vi "remove Line Feed Character.vi"(8 "error in":errorcluster, 11 "Query String":string) -> (0 "error out":errorcluster, 3 "Line Feed Removed String":string)   [LabVIEW 2023, in "ANRITSU Call Box.lvlib"]
uses:
  ANRITSU Call Box.lvlib
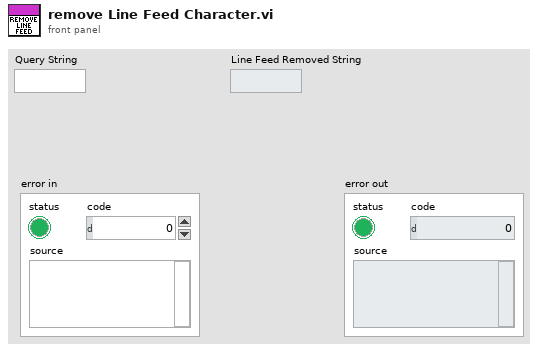
[diagram p1: front panel]
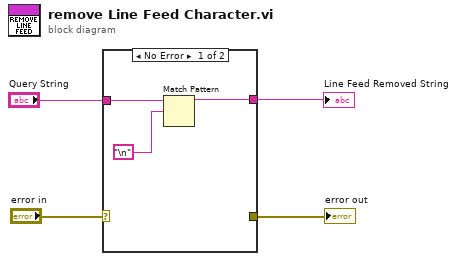
[diagram p0: block diagram]
diagram:
  n1 = case shown="No Error" "error in" {
    selector: "error in" -> [_ w8]
    tunnel: "Query String" -> [w7 _]
    tunnel: [w5 _] -> w3
    tunnel: [_ w8] -> w1
    frame No Error {
      n2 = Match Pattern(string=w7, regular expression="\n") -> (before substring=w5:string)  [unwired: 1 in, 3 out]
    }
    frame Error {
    }
  }
  "Line Feed Removed String" <- w3
  "error out" <- w1
